vi "Read File.vi"(7 "Address":string, 8 "Error In":errorcluster) -> (0 "Error Out":errorcluster)   [LabVIEW 2018, in "Tests.lvlib" / "Known Hosts.lvlib"]
uses:
  Known Hosts.lvlib
  <vilib>/Utility/error.llb/Clear Errors.vi
  src/Toolkit/Known Hosts/Support/Create from Session.vi
  <vilib>/Utility/sysdir.llb/Get System Directory.vi
  src/Toolkit/Known Hosts/Support/Destroy to Session.vi
  <vilib>/addons/_JKI Toolkits/Caraya/classes/Test/Test.lvclass
  <vilib>/addons/_JKI Toolkits/Caraya/classes/Assert/Assert.lvclass
  src/Toolkit/Known Hosts/Known Hosts.lvclass
  Tests.lvlib
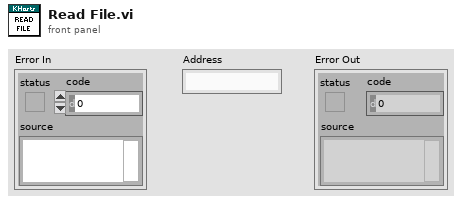
[diagram p1: front panel]
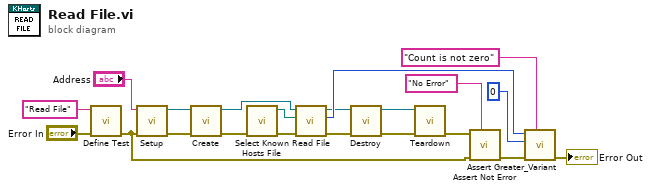
[diagram p0: block diagram]
diagram:
  n1 = call <vilib>:"Define Test.vi"("error in (no error)"="Error In", "Label (VI Title)"="Read File") -> ("error out"=w9:errorcluster)  [unwired: 9 in]
  n2 = call "Setup.vi"("Error In"=w9, "Address In"="Address") -> ("Error Out"=w2:errorcluster, "Sesssion"=w1:refnum<class "Session.lvclass">)  [unwired: 7 in, 1 out]
  n3 = call-poly "Create.vi"("Error In"=w2, "Session"=w1) -> ("Error Out"=w3:errorcluster, "Known Hosts"=w4:refnum<class "Known Hosts.lvclass">)  [unwired: 8 in]
  n4 = call "Select Known Hosts File.vi"("Error In"=w3) -> ("Error Out"=w13:errorcluster, "Known Hosts File"=w12:path)  [unwired: 9 in]
  n5 = call "Read File.vi"("Error In"=w13, "File"=w12, "Known Hosts In"=w4) -> ("Error Out"=w5:errorcluster, "Count"=w16:u64, "Known Hosts Out"=w8:refnum<class "Known Hosts.lvclass">)  [unwired: 6 in]
  n6 = call-poly "Destroy.vi"("Error In"=w5, "Known Hosts"=w8) -> ("Error Out"=w6:errorcluster, "Session"=w7:refnum<class "Session.lvclass">)  [unwired: 8 in]
  n7 = call "Teardown.vi"("Error In"=w6, "Session"=w7) -> ("Error Out"=w11:errorcluster)  [unwired: 9 in]
  n8 = call <vilib>:"Assert Not Error.vi"("Label"="No Error", "error in (no error)"=w9, "Not Error?"=w11) -> ("error out"=w18:errorcluster)  [unwired: 8 in]
  n9 = call <vilib>:"Assert Greater_Variant.vi"("Label"="Count is not zero", "error in (no error)"=w18, "Y"=u64 0 ("Count"), "X"=w16) -> ("error out"=→"Error Out":errorcluster)  [unwired: 7 in]
